vi "Example_Loopback_Check.vi"(8 "error in (no error)":errorcluster, 9 "stats in":T1, 10 "tx id":u32 format="%.0x", 11 "frames":T2 {"flags" format="%.0x"; "id" format="%.0x"}) -> (0 "error out":errorcluster, 1 "stats out":T1)   [LabVIEW 2021]
doc: "Example: for each received frame with ID tx id (not TX ack, not error, = 4 bytes): sequence check (missing += gaps), round-trip time = now - send time of that sequence (µs), min/mean/max."
uses:
  api/CANsub_Channel/CANsub_Channel.lvclass
  api/Typedefs/CANsub_Frames.ctl
  api/CANsub_API.lvlib
  Example_Loopback_Stats.ctl
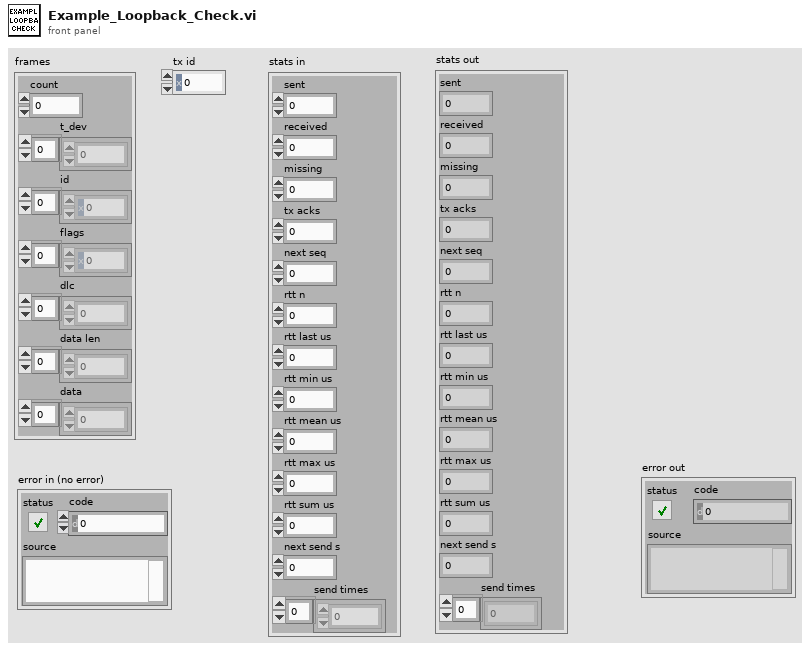
[diagram p1: front panel]
types:
  T1 = typedef "Example_Loopback_Stats.ctl" = cluster{"sent":u32, "received":u32, "missing":u32, "tx acks":u32, "next seq":u32, "rtt n":u32, "rtt last us":dbl, "rtt min us":dbl, "rtt mean us":dbl, "rtt max us":dbl, "rtt sum us":dbl, "next send s":dbl, "send times":dbl[]}
  T2 = typedef "CANsub_API.lvlib/CANsub_Frames.ctl" = cluster{"count":i32, "t_dev":dbl[], "id":u32[], "flags":u16[], "dlc":u8[], "data len":u8[], "data":u8[]}
  T3 = typedef "CANsub_API.lvlib/CANsub_Frame.ctl" = cluster{"id":u32, "t_dev":dbl, "dlc":u8, "data len":u8, "ide":bool, "fdf":bool, "rtr":bool, "brs":bool, "esi":bool, "tx ack":bool, "error frame":bool}
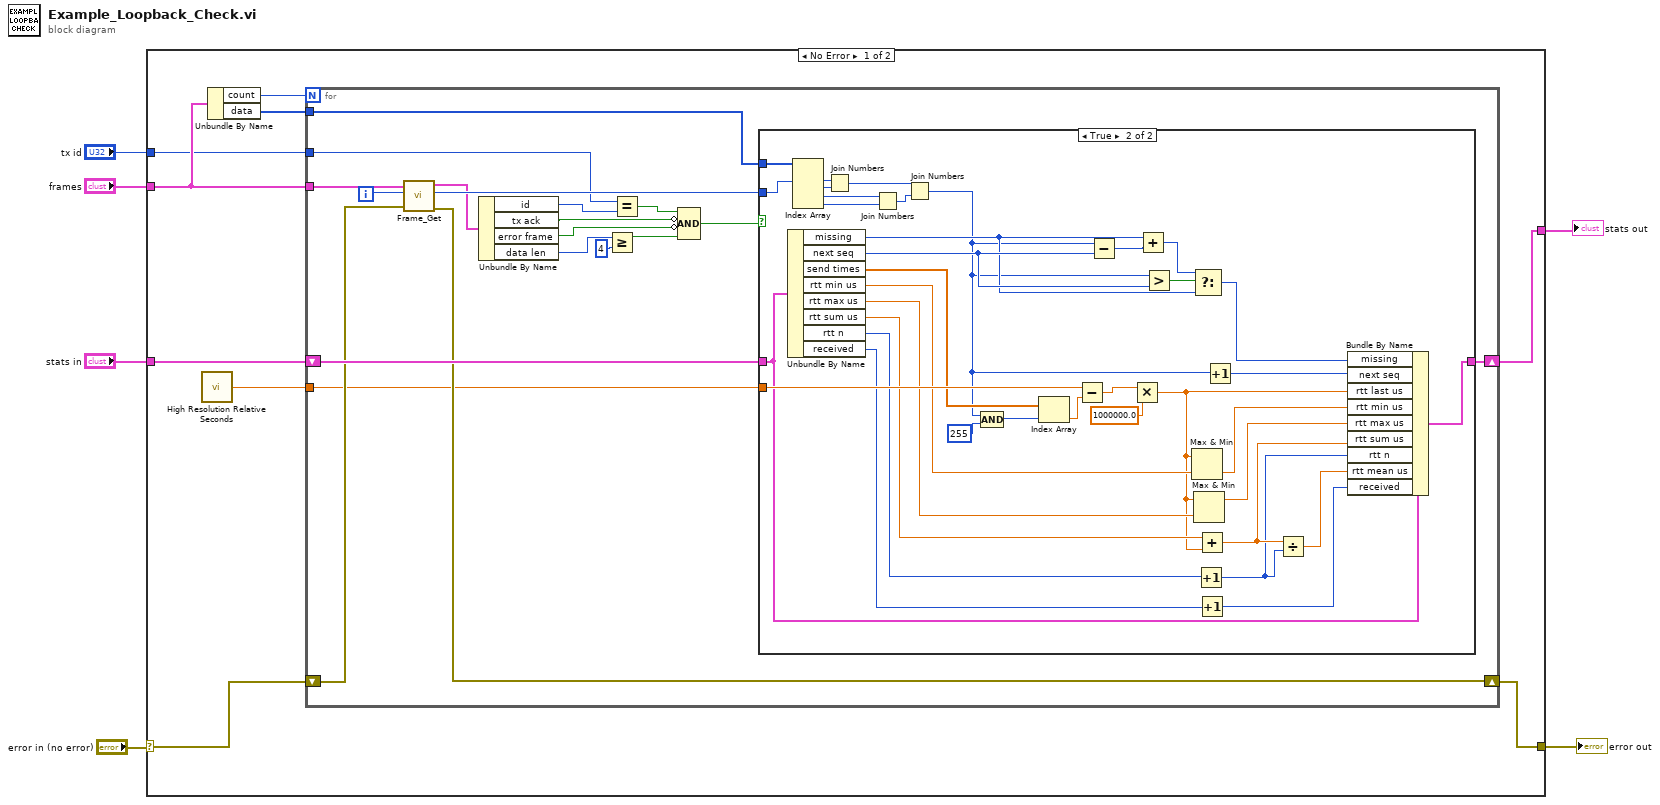
[diagram p0: block diagram]
diagram:
  n1 = case shown="No Error" "error in (no error)" {
    selector: "error in (no error)" -> [w11 w74]
    tunnel: [w7 w74] -> w5
    tunnel: [w12 w73] -> w4
    tunnel: "stats in" -> [w13 w73]
    tunnel: "frames" -> [w15 _]
    tunnel: "tx id" -> [w9 _]
    frame No Error {
      n2 = call <vilib>:"High Resolution Relative Seconds.vi"() -> ("relative seconds"=w8:dbl)
      n3 = Unbundle By Name(w15) -> ("count"=w14:i32, "data"=w10:u8[])
      n4 = for {
        N: w14 -> [_]
        tunnel: w15 -> [w33]
        shift-right: [w31] -> w12
        shift-left: w13 -> [w30]
        shift-right: [w27] -> w7
        shift-left: w11 -> [w28]
        tunnel: w10 -> [w26]
        tunnel: w9 -> [w23]
        tunnel: w8 -> [w16]
        i -> [w34]
        n5 = call "Frame_Get.vi"("error in (no error)"=w28, "i"=w34, "frames"=w33) -> ("error out"=w27:errorcluster, "data offset"=w25:i32, "frame"=w24:T3)  [unwired: 6 in]
        n6 = Unbundle By Name(w24) -> ("id"=w22:u32, "tx ack"=w21:bool, "error frame"=w20:bool, "data len"=w19:u8)
        n7 = Greater Or Equal?(x=w19, y=u8 4) -> (x >= y?=w17:bool)
        n8 = Equal?(x=w23, y=w22) -> (x = y?=w29:bool)
        n9 = Compound Arithmetic op=AND(w29, invert w21, invert w20, w17) -> (w32:bool)
        n10 = case shown="True" w32 {
          tunnel: [w35 w59] -> w31
          tunnel: w30 -> [w35 w60]
          tunnel: w26 -> [_ w72]
          tunnel: w25 -> [_ w71]
          tunnel: w16 -> [_ w64]
          frame False {
          }
          frame True {
            n11 = Unbundle By Name(w60) -> ("missing"=w38:u32, "next seq"=w46:u32, "send times"=w63:dbl[], "rtt min us"=w58:dbl, "rtt max us"=w56:dbl, "rtt sum us"=w54:dbl, "rtt n"=w53:u32, "received"=w49:u32)
            n12 = Index Array(array=w72, index #1=w71) -> (element #1=w70:u8, element #2=w69:u8, element #3=w68:u8, element #4=w67:u8)  [unwired: 3 in]
            n13 = Join Numbers(hi=w70, lo=w69) -> ((hi.lo)=w66:u16)
            n14 = Join Numbers(hi=w68, lo=w67) -> ((hi.lo)=w65:u16)
            n15 = Join Numbers(hi=w66, lo=w65) -> ((hi.lo)=w37:u32)
            n16 = Compound Arithmetic op=AND(w37, u32 255 ("value")) -> (w36:u32)
            n17 = Index Array(array=w63, index=w36) -> (element=w41:dbl)
            n18 = Subtract(x=w64, y=w41) -> (x-y=w40:dbl)
            n19 = Subtract(x=w37, y=w46) -> (x-y=w47:u32)
            n20 = Multiply(x=w40, y=1000000.0) -> (x*y=w39:dbl)
            n21 = Add(x=w38, y=w47) -> (x+y=w44:u32)
            n22 = Greater?(x=w37, y=w46) -> (0:w45:bool)
            n23 = Max & Min(x=w39, y=w58) -> (min(x,y)=w57:dbl)  [unwired: 1 out]
            n24 = Select(t=w44, s=w45, f=w38) -> (s? t:f=w43:u32)
            n25 = Max & Min(x=w39, y=w56) -> (max(x,y)=w55:dbl)  [unwired: 1 out]
            n26 = Increment(x=w53) -> (x+1=w50:u32)
            n27 = Add(x=w54, y=w39) -> (x+y=w52:dbl)
            n28 = Increment(x=w49) -> (x+1=w48:u32)
            n29 = Increment(x=w37) -> (x+1=w42:u32)
            n30 = Divide(x=w52, y=w50) -> (x/y=w51:dbl)
            n31 = Bundle By Name(cluster=w60, "missing"=w43, "next seq"=w42, "rtt last us"=w39, "rtt min us"=w57, "rtt max us"=w55, "rtt sum us"=w52, "rtt n"=w50, "rtt mean us"=w51, "received"=w48) -> (w59:T1)
          }
        }
      }
    }
    frame Error {
    }
  }
  "error out" <- w5
  "stats out" <- w4
